vi "Utility - Convert Filename ICO to PNG.vi"(10 "Convert .ico to .png (T)":bool=TRUE, 11 "Path":path) -> (3 "Path 2":path)   [LabVIEW 2014]
doc: "::: VI Helpeks :::\nCopyright (c) 2000-2026 Konstantin Shifershteyn. All rights reserved."
panel:
  # "VI Helpeks\nCopyright (c) 2012-2026 Konstantin Shifershteyn"
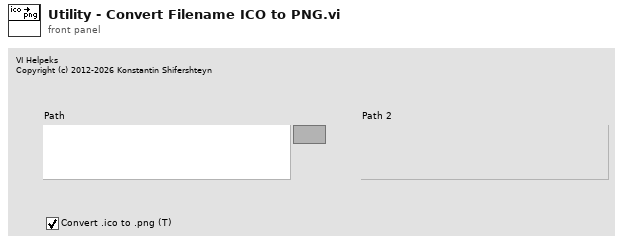
[diagram p1: front panel]
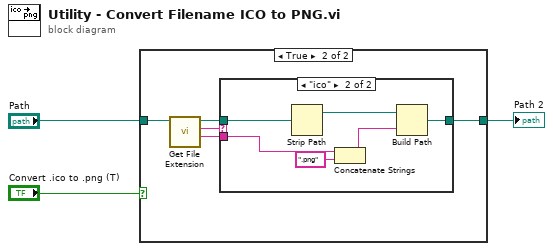
[diagram p0: block diagram]
diagram:
  n1 = case shown="True" "Convert .ico to .png (T)" {
    tunnel: "Path" -> [w4 w9]
    tunnel: [w4 w7] -> w2
    frame False {
    }
    frame True {
      n2 = call <vilib>:"Get File Extension.vi"("file"=w9) -> ("filename without extension"=w5:string, "lowercase file extension"=w8:string, "dup file"=w6:path)  [unwired: 7 in, 1 out]
      n3 = case shown="\"ico\"" w8 {
        tunnel: [w10 w15] -> w7
        tunnel: w6 -> [w10 w16]
        tunnel: w5 -> [_ w13]
        frame Default {
        }
        frame "ico" {
          n4 = Strip Path(path=w16) -> (stripped path=w14:path)  [unwired: 1 out]
          n5 = Concatenate Strings(w13, ".png" ("string")) -> (w11:string)
          n6 = Build Path(base path=w14, name or relative path=w11) -> (appended path=w15:path)
        }
      }
    }
  }
  "Path 2" <- w2
